vi "TeleOp Default.vi"(10 "Occurrence Refnum":refnum<k4>, 11 "OpMode Index":u64 format="%.0x") -> ()   [LabVIEW 2023]
uses:
  <vilib>/MRC/MrcLib.lvlib
  <vilib>/MRC/Types/WPI_JoystickDeviceEnum.ctl
  <vilib>/MRC/Types/XBox Buttons Index.ctl
  af29dd68-2a4b-3fe0-80c6-9da27f27ac3f.vi
  cbb6bf50-7a68-3fe8-201a-3d7722f0bd3f.vi
  <vilib>/MRC/MrcLib/VIs/IMU/IMU Get Yaw Flat.vi
  Robot Global Data.vi
  swerve-template/Type Definitions/Data/Robot Velocities.ctl
  Cascade/Implementation/Cascade Positions.ctl
panel:
  in  "Position":T1
  in  "x":T2={"X Velocity"=5.0, "Y Velocity"=5.0, "Rotational \nVelocity"=180.0}
  out "RobotMode":u8
  out "Match Time(s)":sgl
  # "Do not rename these\ntwo controls"
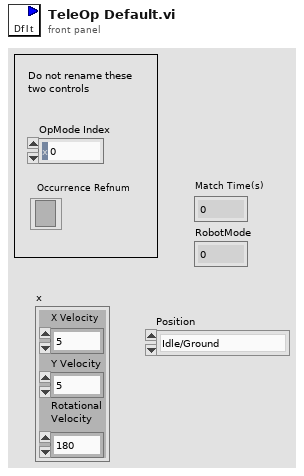
[diagram p1: front panel]
types:
  T1 = typedef "Cascade Positions.ctl" = enum16{"Idle/Ground", "Raised L1", "L2", "L2 Tip", "L3", "L3 Tip", "Feeder", "\"Default\""}
  T2 = typedef "Robot Velocities.ctl" = cluster{"X Velocity":dbl, "Y Velocity":dbl, "Rotational \nVelocity":dbl}
  T3 = typedef "XBox Buttons Index.ctl" = enum16{"A", "B", "X", "Y", "Back", "Logo", "Start", "Left Joystick", "Right Joystick", "Left Bumper", "Right Bumper"}
  T4 = typedef "WPI_JoystickDeviceEnum.ctl" = enum16{"USB 0", "USB 1", "USB 2", "USB 3", "USB 4", "USB 5"}
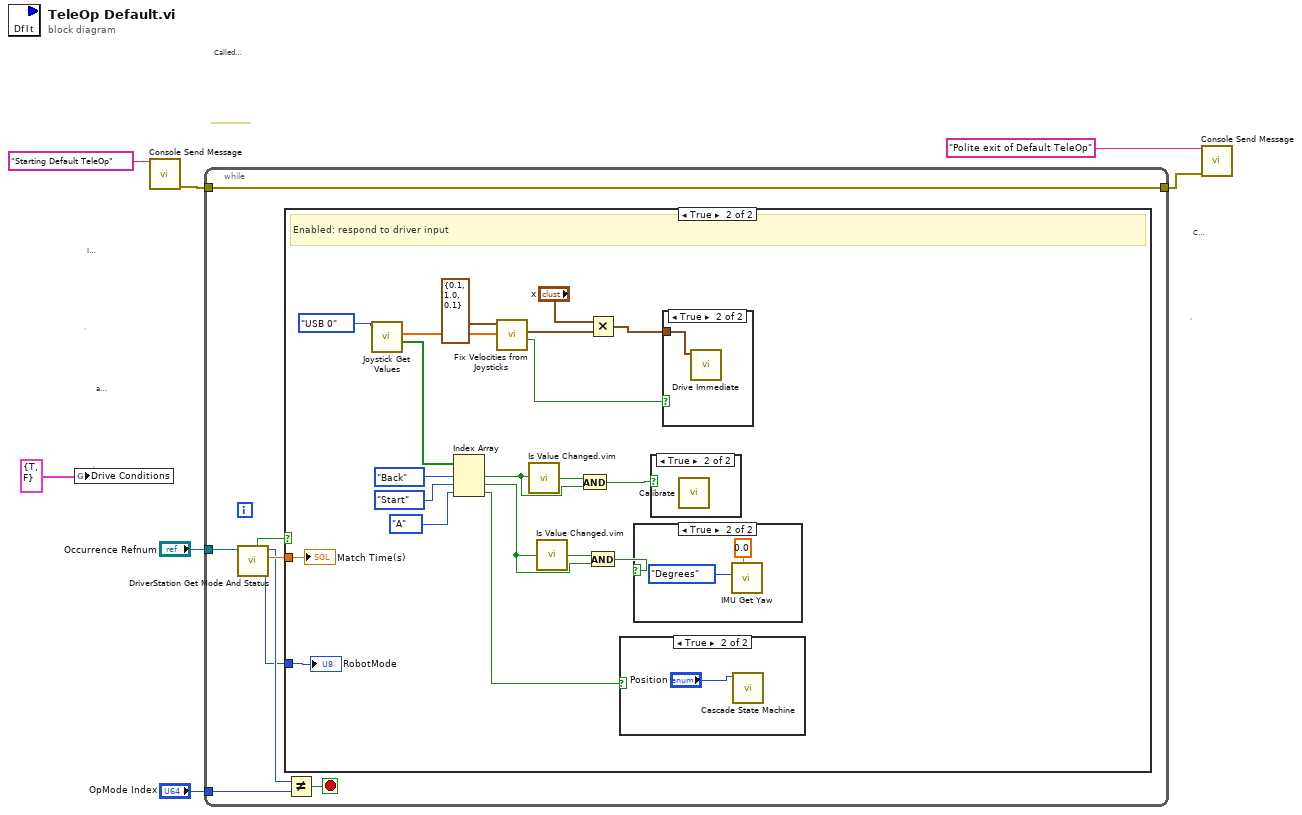
[diagram p0: block diagram]
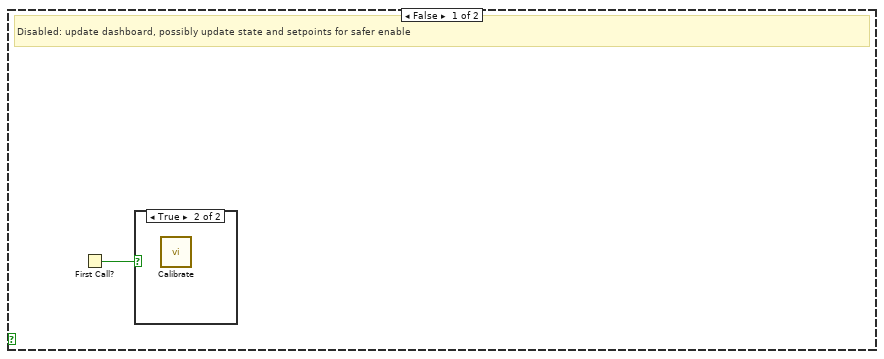
[diagram p2: hidden frame]
diagram:
  # "add enabled counter\nstats, etc"
  # "Cleanup I/O"
  # "Called once when teleOp is selected by DS.\nLoop until mode changes carrying out enabled\nor disabled response."
  # "Init I/O and anything\nused during TeleOp"
  n1 = global write "Robot Global Data.vi" "Drive Conditions"(cluster{"Field Centric":bool, "Reset PIDs":bool} {"Field Centric"=TRUE, "Reset PIDs"=FALSE} ("Drive Conditions")) -> ()
  n2 = call <vilib>:"Console Send Message.vi"("Message"="Starting Default TeleOp") -> ("error out"=w5:errorcluster)  [unwired: 14 in]
  n3 = while {
    tunnel: "OpMode Index" -> [w13]
    tunnel: [w9] -> w3
    tunnel: w5 -> [w9]
    tunnel: "Occurrence Refnum" -> [w8]
    stop <- w12 stop-if-true
    n4 = call <vilib>:"DriverStation Get Mode And Status.vi"("Occurrence Refnum"=w8) -> ("RobotMode"=w10:u8, "Match Time(s)"=w15:sgl, "currentOpMode"=w11:u64, "Enabled"=w14:bool)  [unwired: 5 in, 2 out]
    n5 = case shown="True" w14 {
      tunnel: w15 -> [_ w36]
      tunnel: w10 -> [_ w35]
      frame False {
        # "Disabled: update dashboard, possibly update state and setpoints for safer enable"
        n6 = First Call?() -> (First Call?: T/F=w16:bool)
        n7 = case shown="True" w16 {
          frame False {
          }
          frame True {
            n8 = call "Calibrate.vi"() -> ()  [unwired: 11 in, 1 out]
          }
        }
      }
      frame True {
        # "Enabled: respond to driver input"
        n9 = call <vilib>:"Joystick Get Values.vi"("Joystick"=WPI_JoystickDeviceEnum."USB 0") -> ("Buttons"=w27:bool[], "Axes"=w33:dbl[])  [unwired: 5 in, 4 out]
        n10 = Index Array(array=w27, index #1=XBox_Buttons_Index."Back" ("XBox Buttons"), index #2=XBox_Buttons_Index."Start" ("XBox Buttons"), index #3=XBox_Buttons_Index."A" ("XBox Buttons")) -> (element #1=w24:bool, element #2=w21:bool, element #3=w17:bool)
        n11 = call "Fix Velocities from Joysticks.vi"("Axes"=w33, "Deadband"=cluster{"value":dbl, "value":dbl, "value":dbl} {"value"=0.1, "value"=1.0, "value"=0.1}) -> ("Sending Input?"=w31:bool, "Adjusted Robot Velocities"=w30:T2)  [unwired: 8 in]
        n12 = call "Is Value Changed.vim"("value"=w24) -> ("changed or first call?"=w25:bool)
        n13 = call "Is Value Changed.vim"("value"=w21) -> ("changed or first call?"=w22:bool)
        n14 = And(x=w25, y=w24) -> (x .and. y?=w23:bool)
        n15 = Multiply(x="x", y=w30) -> (x*y=w29:T2)
        n16 = And(x=w22, y=w21) -> (x .and. y?=w19:bool)
        n17 = case shown="True" w17 {
          frame False {
          }
          frame True {
            n18 = call "Cascade State Machine.vi"("Position"="Position") -> ()  [unwired: 10 in, 1 out]
          }
        }
        n19 = case shown="True" w19 {
          frame False {
          }
          frame True {
            n20 = call-poly <vilib>:"IMU Get Yaw.vi"("Alignment Angle"=0.0, "Units"=enum16{"Radians", "Degrees"}."Degrees") -> ()  [unwired: 7 in, 3 out]
          }
        }
        n21 = case shown="True" w23 {
          frame False {
          }
          frame True {
            n22 = call "Calibrate.vi"() -> ()  [unwired: 11 in, 1 out]
          }
        }
        n23 = case shown="True" w31 {
          tunnel: w29 -> [_ w40]
          frame False {
          }
          frame True {
            n24 = call "Drive Immediate.vi"("Robot Velocities"=w40) -> ()  [unwired: 10 in, 1 out]
          }
        }
        "Match Time(s)" <- w36
        "RobotMode" <- w35
      }
    }
    n25 = Not Equal?(x=w11, y=w13) -> (x != y?=w12:bool)
  }
  n26 = call <vilib>:"Console Send Message.vi"("Message"="Polite exit of Default TeleOp", "error in (no error)"=w3) -> ()  [unwired: 13 in, 1 out]
